vi "Array Ops Probe.vi"() -> ()   [LabVIEW 2026]
doc: "Round6 Task3 probe: array operation node coverage in AIXML. Expected: Arr 123=[1,2,3], Concat=[10,20,30], Indexed=20, Size=3, Subset=[20,30], Inserted=[99,10,20,30], Deleted=[10], Deleted Portion=[20,30], Initialized=[7,7,7], Search Found=2."
panel:
  out "Search Found":i32
  out "Initialized":i32[](array[numeric])
  out "Deleted Portion":i32[](array[numeric])
  out "Deleted":i32[](array[numeric])
  out "Inserted":i32[](array[numeric])
  out "Subset":i32[](array[numeric])
  out "Size":i32
  out "Indexed":i32
  out "Concat":i32[](array[numeric])
  out "Arr 123":i32[](array[numeric])
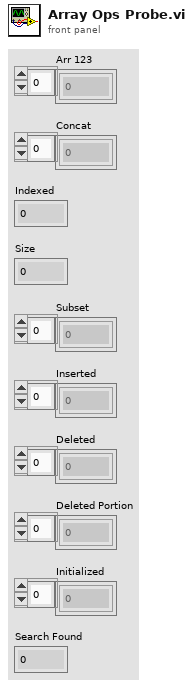
[diagram p1: front panel]
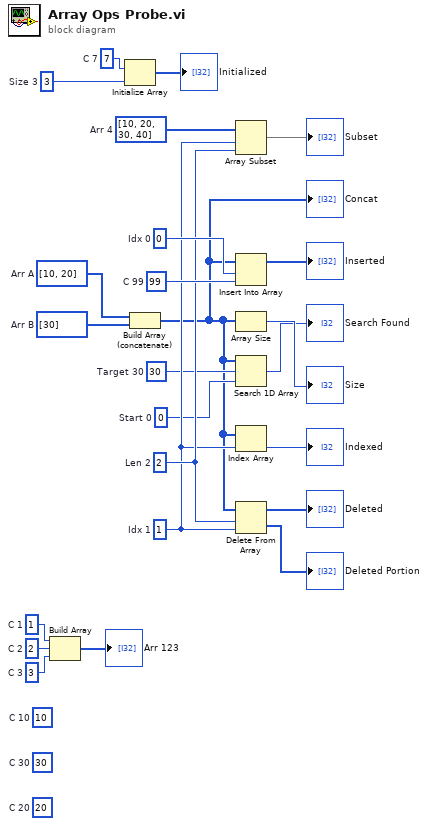
[diagram p0: block diagram]
diagram:
  w11 = 0  # Start 0
  w12 = 30  # Target 30
  w13 = 3  # Size 3
  w18 = 0  # Idx 0
  w16 = 2  # Len 2
  w15 = 1  # Idx 1
  w19 = i32[] [10, 20, 30, 40]  # Arr 4
  w20 = i32[] [30]  # Arr B
  w21 = i32[] [10, 20]  # Arr A
  w14 = 7  # C 7
  w17 = 99  # C 99
  (unwired) 30  # C 30
  (unwired) 20  # C 20
  (unwired) 10  # C 10
  w22 = 3  # C 3
  w23 = 2  # C 2
  w24 = 1  # C 1
  n1 = Build Array(w24, w23, w22) -> (→"Arr 123":i32[])
  n2 = Initialize Array(w14, w13) -> (→"Initialized":i32[])
  n3 = Build Array (concatenate)(w21, w20) -> (w9:i32[])
  "Concat" <- w9
  n4 = Array Subset(array=w19, index=w15, length=w16) -> (→"Subset":i32[])
  n5 = Insert Into Array(array=w9, index=w18, new element=w17) -> (→"Inserted":i32[])
  n6 = Array Size(array=w9) -> (size(s)=→"Size":i32)
  n7 = Search 1D Array(1D array=w9, element=w12, start index (0)=w11) -> (index of element=→"Search Found":i32)
  n8 = Index Array(array=w9, index=w15) -> (element=→"Indexed":i32)
  n9 = Delete From Array(array=w9, length=w16, index=w15) -> (deleted portion=→"Deleted Portion":i32[], array with subset deleted=→"Deleted":i32[])
